vi "RemoteVI Click State.vi"(0 "popups out":T1, 1 "recent click?":bool, 2 "popup open?":bool, 5 "clicked?":bool, 7 "now":u32, 9 "last click":u32) -> (4 "d":cluster{"dx":i32, "dy":i32}, 6 "last click out":u32, 8 "no VI Server?":bool)   [LabVIEW 2020, in "RemoteVI.lvlib"]
doc: "The state the server loop keeps after servicing the clients: d (dx, dy of popups out - the displacement a popup click used, for the next iteration); last click out (now when a client posted a message that may open a popup in this iteration, else last click); and no VI Server? - TRUE while a popup is open, a click is recent or happened in this iteration: the loop then makes no VI Server UI call (a popup that is still opening must not catch FP.Get Image in its modal loop). Pure."
uses:
  RemoteVI.lvlib
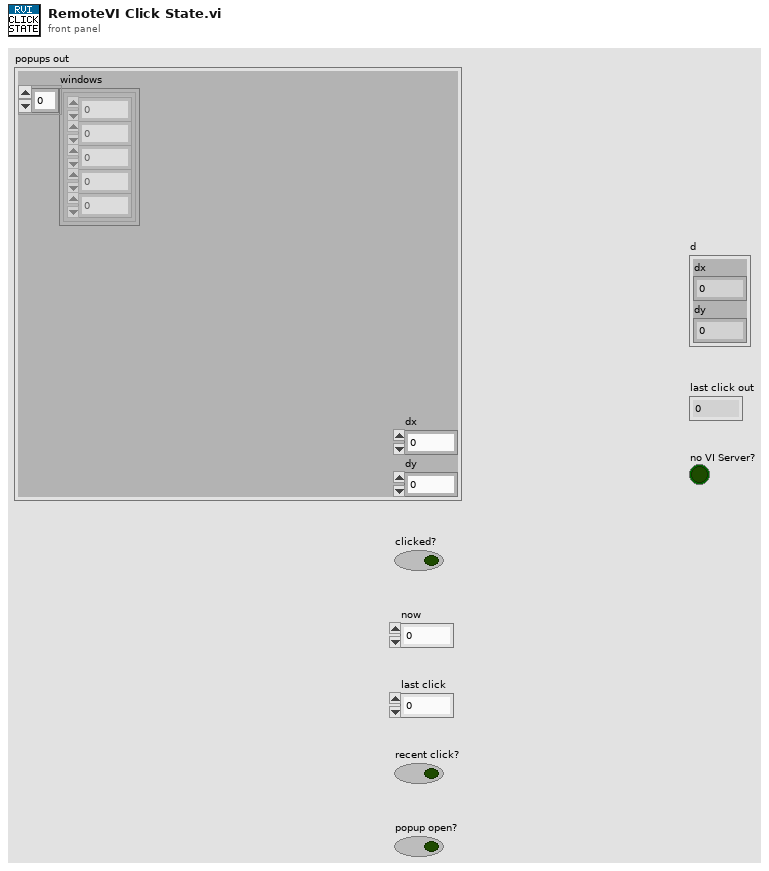
[diagram p1: front panel]
types:
  T1 = cluster{"windows":cluster{"hwnd":u64, "x":i32, "y":i32, "w":i32, "h":i32}[], "dx":i32, "dy":i32}
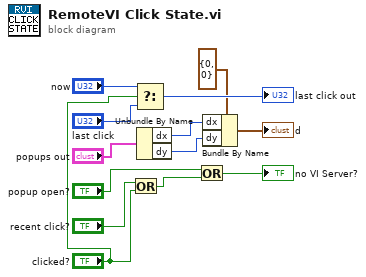
[diagram p0: block diagram]
diagram:
  n1 = Or(x="recent click?", y="clicked?") -> (x .or. y?=w12:bool)
  n2 = Select(t="now", s="clicked?", f="last click") -> (s? t:f=→"last click out":u32)
  n3 = Unbundle By Name("popups out") -> ("dx"=w7:i32, "dy"=w8:i32)
  n4 = Or(x="popup open?", y=w12) -> (x .or. y?=→"no VI Server?":bool)
  n5 = Bundle By Name(cluster=cluster{"dx":i32, "dy":i32} {"dx"=0, "dy"=0}, "dx"=w7, "dy"=w8) -> (→"d":cluster{"dx":i32, "dy":i32})
